vi "Recurse Cluster or Array.vi"(8 "Skip Outer Cluster":bool, 9 "Cluster or Array":variant, 10 "Lookup String":string, 11 "PropertyObject":refnum<k7>) -> (0 "error out":errorcluster)   [LabVIEW 2020, in "TSS.lvlib" / "VariableContainer.lvclass"]
uses:
  VariableContainer.lvclass
  <vilib>/Negentropic/Serializable/Property Bag/Property Bag.lvclass
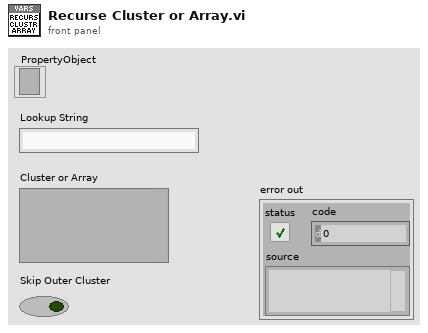
[diagram p1: front panel]
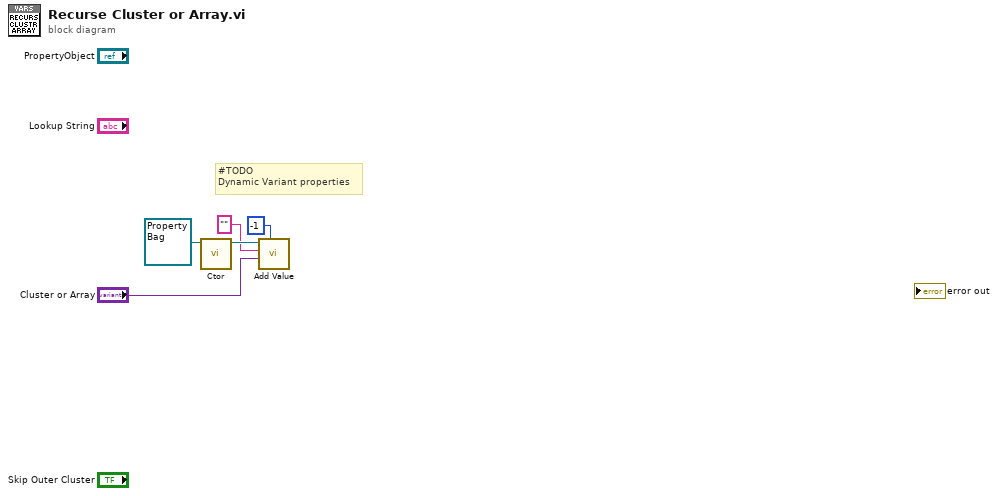
[diagram p0: block diagram]
diagram:
  # "#TODO\nDynamic Variant properties"
  n1 = call-dynamic "Ctor.vi"("Property Bag In"=refnum<class "Property Bag.lvclass"> refnum ("Property Bah In")) -> ("Property Bag out"=w5:refnum<class "Property Bag.lvclass">)  [unwired: 9 in, 1 out]
  n2 = call <vilib>:"Add Value.vi"("Parent Index"=-1, "Value"="Cluster or Array", "Name"="", "Property Bag in"=w5) -> ()  [unwired: 5 in, 3 out]
